vi "Insert Into Subpanel.vi"(8 "error in (no error)":errorcluster, 11 "Data in":T1={"PeekVI Reference"=refnum, "SubPanel"=refnum, "Peek Stack Tree Ref"=refnum, "Open Button Ref"=refnum, "Top VI"=refnum, "Active VI"=refnum, "Stack"=[], "Last FP State"=enum."Standard"}) -> (0 "error out":errorcluster, 3 "Data out":T1={"PeekVI Reference"=refnum, "SubPanel"=refnum, "Peek Stack Tree Ref"=refnum, "Open Button Ref"=refnum, "Top VI"=refnum, "Active VI"=refnum, "Stack"=[], "Last FP State"=enum."Standard"})   [LabVIEW 2020, in "Peek Window.lvlib"]
uses:
  Peek Window.lvlib
  MHL Data Cluster.ctl
  VI Types/Standard VI Type/Standard VI Type.lvclass
  VI Types/Standard VI Type/Standard VI Type.lvclass/Standard VI Type.ctl
  VI Types/Standard VI Type/Read Openable.vi
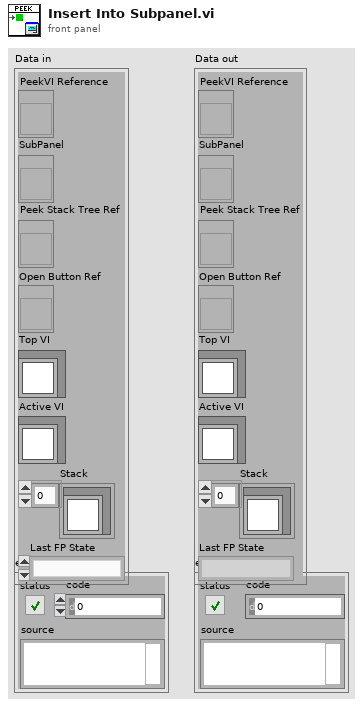
[diagram p1: front panel]
types:
  T1 = typedef "Peek Window.lvlib/MHL Data Cluster.ctl" = cluster{"PeekVI Reference":refnum<vi>, "SubPanel":refnum<vi>, "Peek Stack Tree Ref":refnum<vi>, "Open Button Ref":refnum<vi>, "Top VI":refnum<class "Standard VI Type.lvclass">, "Active VI":refnum<class "Standard VI Type.lvclass">, "Stack":refnum<class "Standard VI Type.lvclass">[], "Last FP State":enum32{"Invalid", "Standard", "Closed", "Hidden", "Minimized", "Maximized"}}
  T2 = enum8{"Enabled", "Disabled", "Disabled and Grayed Out"}
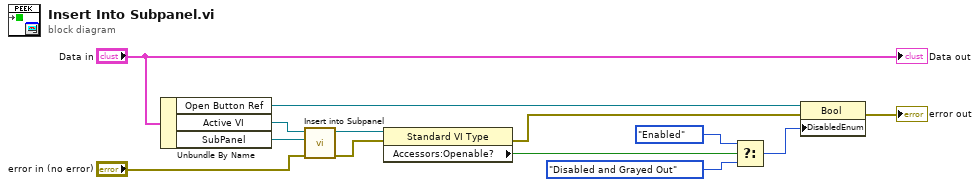
[diagram p0: block diagram]
diagram:
  n1 = Unbundle By Name("Data in") -> ("Open Button Ref"=w9:refnum<vi>, "Active VI"=w11:refnum<class "Standard VI Type.lvclass">, "SubPanel"=w12:refnum<vi>)
  n2 = call-dynamic "Insert into Subpanel.vi"("error in (no error)"="error in (no error)", "SubPanel"=w12, "Standard VI Type in"=w11) -> ("error out"=w7:errorcluster, "Standard VI Type out"=w8:refnum<class "Standard VI Type.lvclass">)  [unwired: 7 in]
  n3 = property class="Standard VI Type"(reference=w8, error in=w7) -> (error out=w2:errorcluster, "Accessors:Openable?"=w6:bool)  [unwired: 1 out]
  n4 = Select(t=T2."Enabled", s=w6, f=T2."Disabled and Grayed Out") -> (s? t:f=w3:T2)
  n5 = property class="Bool"(reference=w9, error in=w2, "DisabledEnum"=w3) -> (error out=→"error out":errorcluster)  [unwired: 1 out]
  "Data out" <- "Data in"
